vi "Utilization Test.vi"() -> ()   [LabVIEW 2019]
uses:
  Asset External Calibration/Asset External Calibration.lvclass
  <vilib>/Skyline/AssetManagement/Start Utilization (All).vi
  <vilib>/Skyline/AssetManagement/Start Utilization (Single).vi
  Asset/Asset.lvclass
  <vilib>/Skyline/AssetManagement/NI SystemLink Asset Utilization.lvclass
  <vilib>/Skyline/Utilities/NI Skyline Utilities.lvlib
panel:
  out "Utilizations":i32
  in  "Number of assets":i32=10
  out "Assets":string[](array[string])
  out "Iteration":i32
  in  "stop":bool
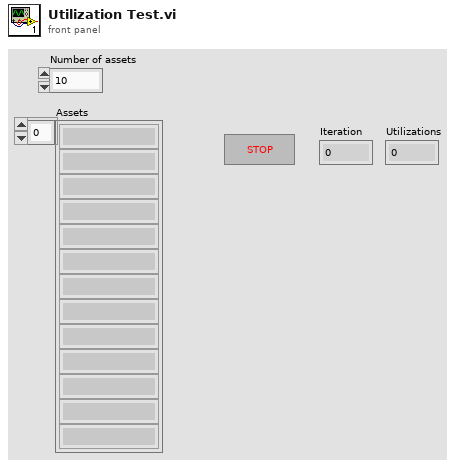
[diagram p1: front panel]
types:
  T1 = enum16{"BuiltInSystem", "PciPxi", "Usb", "Gpib", "Vxi", "Serial", "TcpIp", "cRio", "Scxi", "cDaq", "SwitchBlock", "Scc", "FireWire", "Accessory", "Can", "SwitchBlockDevice"}
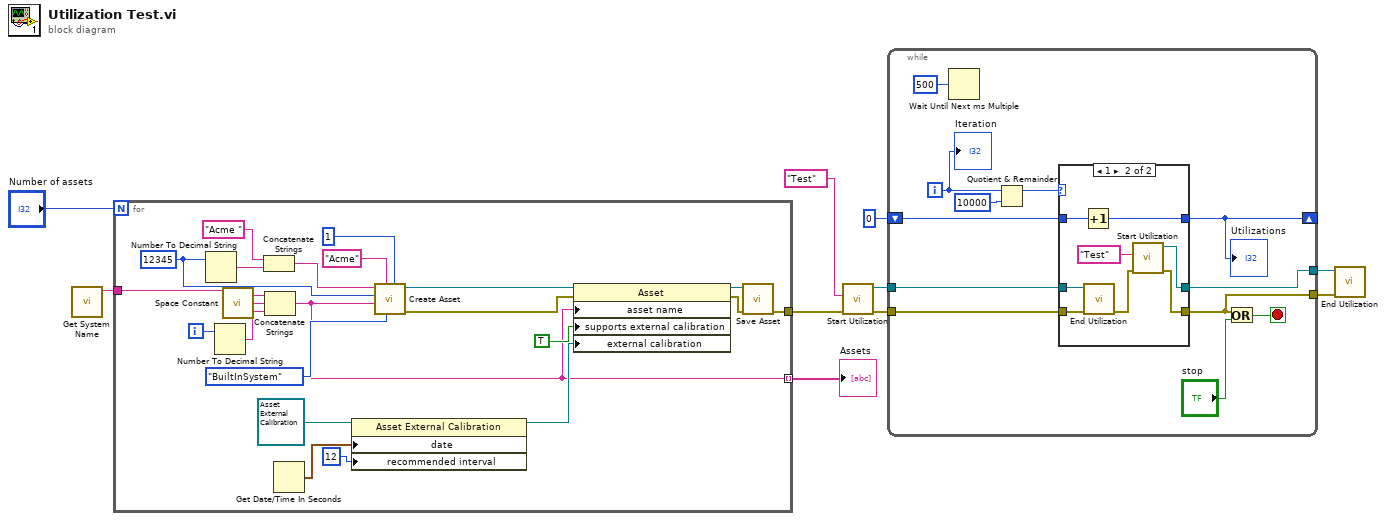
[diagram p0: block diagram]
diagram:
  n1 = call <vilib>:"Get System Name.vi"() -> ("system name"=w3:string)  [unwired: 11 in]
  n2 = for {
    N: "Number of assets" -> [_]
    tunnel: [w30] -> w6
    tunnel: w3 -> [w18]
    tunnel: [w11] -> w2 mode=indexing
    i -> [w17]
    w15 = u32 12345 ("Model Number")
    n3 = Number To Decimal String(number=w15) -> (decimal integer string=w13:string)  [unwired: 1 in]
    n4 = Number To Decimal String(number=w17) -> (decimal integer string=w16:string)  [unwired: 1 in]
    n5 = call <vilib>:"Space Constant.vi"() -> ("String"=w14:string)
    n6 = Concatenate Strings("Acme " ("Model Name"), w13) -> (w12:string)
    n7 = Concatenate Strings(w18, w14, w16) -> (w11:string)
    n8 = Get Date/Time In Seconds() -> (seconds since 1Jan1904=w20:timestamp)
    n9 = property class="Asset External Calibration"(reference=refnum<class "Asset External Calibration.lvclass"> refnum ("external calibration"), "date"=w20, "recommended interval"=u32 12) -> (reference out=w21:refnum<class "Asset External Calibration.lvclass">)  [unwired: 1 in, 1 out]
    n10 = call "Create Asset.vi"("Vendor Number"=u32 1, "Bus Type"=T1."BuiltInSystem", "Vendor Name"="Acme", "Serial Number"=w11, "Model Number"=w15, "Model Name"=w12) -> ("Error Out"=w28:errorcluster, "Asset"=w25:refnum<class "Asset.lvclass">)  [unwired: 4 in]
    n11 = property class="Asset"(reference=w25, error in=w28, "asset name"=w11, "supports external calibration"=TRUE, "external calibration"=w21) -> (reference out=w26:refnum<class "Asset.lvclass">, error out=w27:errorcluster)
    n12 = call "Save Asset.vi"("Error In"=w27, "Asset"=w26) -> ("Error Out"=w30:errorcluster)  [unwired: 9 in]
  }
  "Assets" <- w2
  n13 = call-poly <vilib>:"Start Utilization.vi"("error in (no error)"=w6, "utilization category"="Test") -> ("error out"=w9:errorcluster, "asset utilization"=w10:refnum<class "NI SystemLink Asset Utilization.lvclass">)  [unwired: 8 in]
  n14 = while {
    tunnel: [w35] -> w7
    tunnel: w10 -> [w38]
    tunnel: w9 -> [w37]
    tunnel: [w36] -> w8
    shift-right: [w33] -> _
    shift-left: 0 -> [w34]
    i -> [w41]
    stop <- w42 stop-if-true
    n15 = Wait Until Next ms Multiple(millisecond multiple=u32 500) -> ()  [unwired: 1 out]
    n16 = Quotient & Remainder(x=w41, y=10000) -> (x-y*floor(x/y)=w39:i32)  [unwired: 1 out]
    n17 = case shown="1" w39 {
      tunnel: w38 -> [w47 w54]
      tunnel: w37 -> [w46 w53]
      tunnel: [w46 w52] -> w36
      tunnel: [w47 w51] -> w35
      tunnel: w34 -> [w45 w49]
      tunnel: [w45 w48] -> w33
      frame 0, Default {
      }
      frame 1 {
        n18 = Increment(x=w49) -> (x+1=w48:i32)
        n19 = call <vilib>:"End Utilization.vi"("error in (no error)"=w53, "asset utilization"=w54) -> ("error out"=w55:errorcluster)  [unwired: 9 in]
        n20 = call-poly <vilib>:"Start Utilization.vi"("error in (no error)"=w55, "utilization category"="Test") -> ("error out"=w52:errorcluster, "asset utilization"=w51:refnum<class "NI SystemLink Asset Utilization.lvclass">)  [unwired: 8 in]
      }
    }
    "Utilizations" <- w33
    n21 = Or(x=w36, y="stop") -> (x .or. y?=w42:bool)
    "Iteration" <- w41
  }
  n22 = call <vilib>:"End Utilization.vi"("error in (no error)"=w8, "asset utilization"=w7) -> ()  [unwired: 9 in, 1 out]
